vi "TrajectoryUtil_toPathWeaverJSON.vi"(7 "AlwaysOverWrite":bool, 8 "error in (no error)":errorcluster, 10 "inTRAJECTORY":T1 {"States"."POSE"."ROTATION"."SIN" format="%13.4f"; "States"."POSE"."ROTATION"."COS" format="%13.4f"; "States"."POSE"."ROTATION"."VALUE" format="%13.4f"; "States"."POSE"."TRANSLATION"."Y" format="%14.3f"; "States"."POSE"."TRANSLATION"."X" format="%14.3f"; "TotalTImeSecs" format="%20.3f"}, 11 "FileName":string="trajectory.json") -> (0 "error out":errorcluster, 4 "Full Filename":string)   [LabVIEW 2019, in "Trajectory_Library.lvlib"]
doc: "Exports a Trajectory to a PathWeaver-style JSON file.\n\nParameters:\n - Always Overwrite -- This optional terminal, if TRUE, will not prompt on WINDOWS to overwrite an existing file. On the RoboRIO the file is always overwritten. ( Default: False )\n - Trajectory - Trajectory data structure\n - FileName - File name string of the export json file\n - Error In - Error cluster (not used)\n\nReturns:\n - Error out - Returned error cluster"
uses:
  Trajectory_Library.lvlib
  TypeDef/TRAJECTORY.ctl
  TypeDef/TRAJ_STATE.ctl
  TypeDef/POSE2D.ctl
  TypeDef/TRANSLATION2D.ctl
  TypeDef/ROTATION2D.ctl
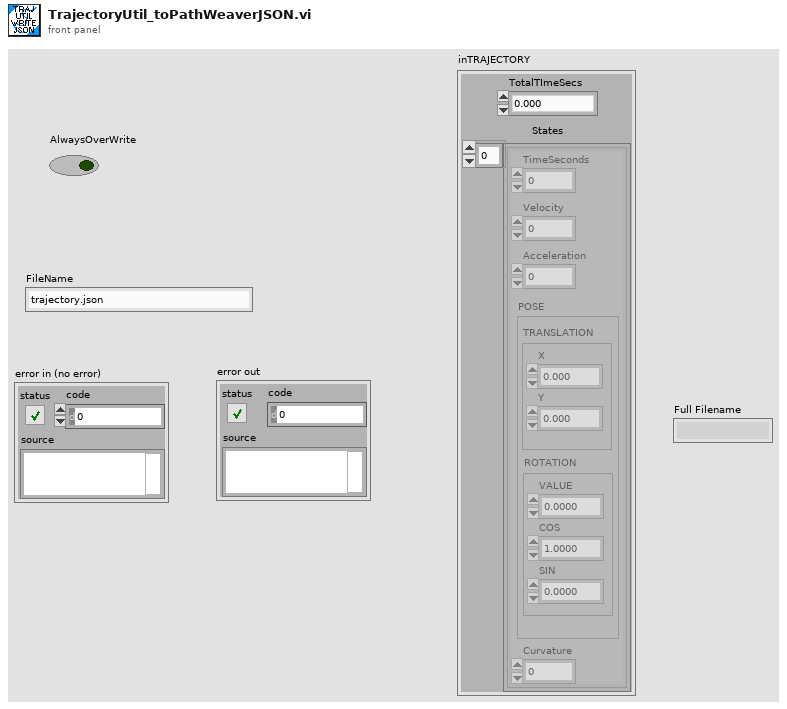
[diagram p1: front panel]
types:
  T1 = typedef "Trajectory_Library.lvlib/TRAJECTORY.ctl" = cluster{"TotalTImeSecs":dbl, "States":T2[]}
  T2 = typedef "Trajectory_Library.lvlib/TRAJ_STATE.ctl" = cluster{"TimeSeconds":dbl, "Velocity":dbl, "Acceleration":dbl, "POSE":T3, "Curvature":dbl}
  T3 = typedef "Trajectory_Library.lvlib/POSE2D.ctl" = cluster{"TRANSLATION":T4, "ROTATION":T5}
  T4 = typedef "Trajectory_Library.lvlib/TRANSLATION2D.ctl" = cluster{"X":dbl, "Y":dbl}
  T5 = typedef "Trajectory_Library.lvlib/ROTATION2D.ctl" = cluster{"VALUE":dbl, "COS":dbl, "SIN":dbl}
  T6 = enum16{"open", "replace", "create", "open or create", "replace or create", "replace or create with confirmation"}
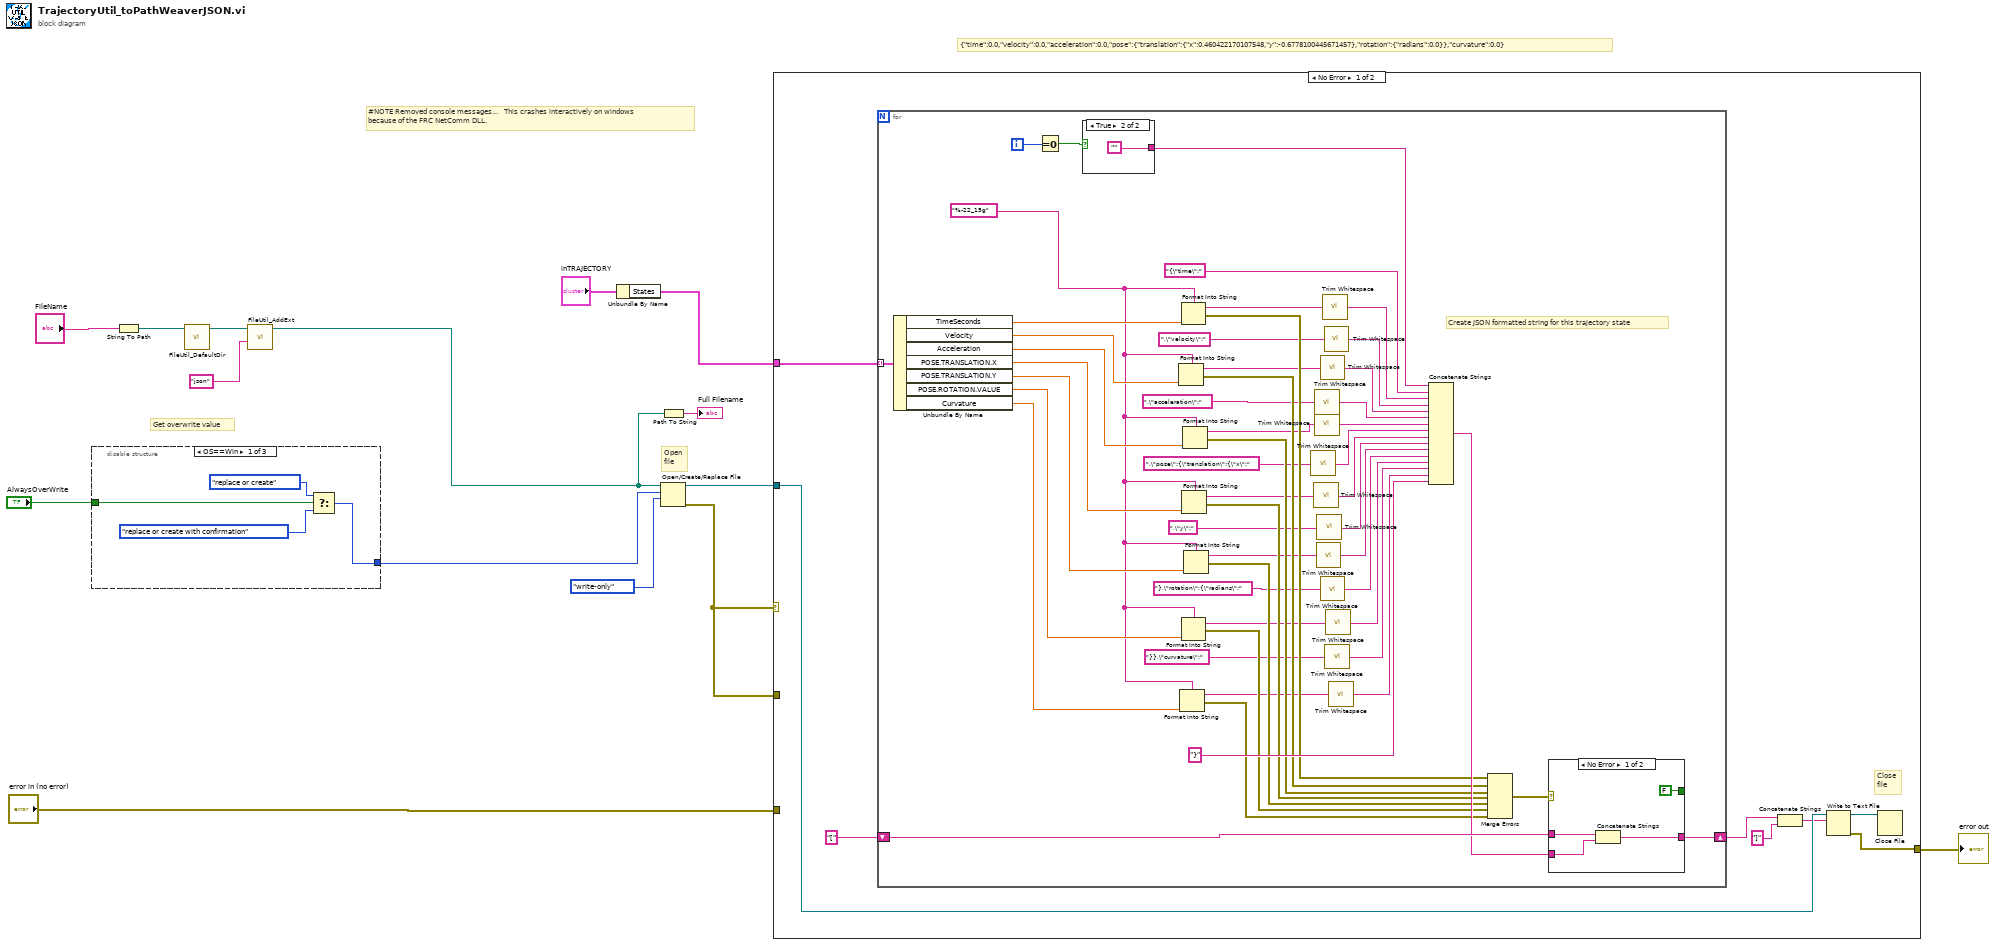
[diagram p0: block diagram]
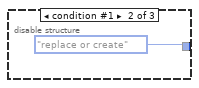
[diagram p2: hidden frame]
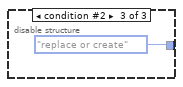
[diagram p3: hidden frame]
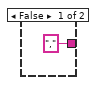
[diagram p4: hidden frame]
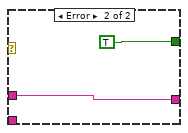
[diagram p5: hidden frame]
diagram:
  # "Get overwrite value"
  # "#NOTE Removed console messages...   This crashes interactively on windows \nbecause of the FRC NetComm DLL."
  # "{\"time\":0.0,\"velocity\":0.0,\"acceleration\":0.0,\"pose\":{\"translation\":{\"x\":0.460422170107548,\"y\":-0.6778100445671457},\"rotation\":{\"radians\":0.0}},\"curvature\":0.0}"
  # "Open\nfile"
  n1 = disable-structure shown="OS==Win" {
    disable-tunnel: [w16 T6."replace or create" ("operation (0:open)") T6."replace or create" ("operation (0:open)")] -> w8
    disable-tunnel: "AlwaysOverWrite" -> [w19 _ _]
    frame condition #0 (active) {
      n2 = Select(t=T6."replace or create" ("operation (0:open)"), s=w19, f=T6."replace or create with confirmation" ("operation (0:open)")) -> (s? t:f=w16:T6)
    }
    frame condition #1 {
    }
    frame condition #2 {
    }
  }
  n3 = String To Path(string="FileName") -> (path=w2:path)
  n4 = call "FileUtil_DefaultDir.vi"("Path in"=w2) -> ("Path Out"=w4:path)  [unwired: 10 in]
  n5 = call "FileUtil_AddExt.vi"("Extension"="json", "Path in"=w4) -> ("Path out"=w1:path)  [unwired: 9 in]
  n6 = Unbundle By Name("inTRAJECTORY") -> ("States"=w10:T2[])
  n7 = Open/Create/Replace File(file path (use dialog)=w1, operation (0:open)=w8, access (0:read/write)=enum16{"read/write", "read-only", "write-only"}."write-only") -> (refnum out=w9:refnum<file>, error out=w14:errorcluster)  [unwired: 3 in, 1 out]
  n8 = Path To String(path=w1) -> (string=→"Full Filename":string)
  n9 = case shown="No Error" w14 {
    tunnel: w14 -> [_ w89]
    tunnel: [w23 w89] -> w13
    tunnel: w10 -> [w29 _]
    tunnel: w9 -> [w25 _]
    tunnel: "error in (no error)" -> [_ _]
    frame No Error {
      # "Close\nfile"
      n10 = for {
        tunnel: w29 -> [w79] mode=indexing
        shift-right: [w65] -> w27
        shift-left: "[" -> [w66]
        i -> [w78]
        w56 = "%-22_15g"
        # "Create JSON formatted string for this trajectory state"
        n11 = Unbundle By Name(w79) -> ("TimeSeconds"=w73:dbl, "Velocity"=w72:dbl, "Acceleration"=w71:dbl, "POSE.TRANSLATION.X"=w70:dbl, "POSE.TRANSLATION.Y"=w69:dbl, "POSE.ROTATION.VALUE"=w68:dbl, "Curvature"=w67:dbl)
        n12 = Equal To 0?(x=w78) -> (x = 0?=w77:bool)
        n13 = case shown="True" w77 {
          tunnel: ["," ""] -> w76
          frame False {
          }
          frame True {
          }
        }
        n14 = Format Into String(format string=w56, w72) -> (resulting string=w51:string, error out=w62:errorcluster)  [unwired: 2 in]
        n15 = Format Into String(format string=w56, w67) -> (resulting string=w31:string, error out=w57:errorcluster)  [unwired: 2 in]
        n16 = Format Into String(format string=w56, w73) -> (resulting string=w55:string, error out=w63:errorcluster)  [unwired: 2 in]
        n17 = Format Into String(format string=w56, w68) -> (resulting string=w35:string, error out=w58:errorcluster)  [unwired: 2 in]
        n18 = Format Into String(format string=w56, w70) -> (resulting string=w43:string, error out=w60:errorcluster)  [unwired: 2 in]
        n19 = Format Into String(format string=w56, w71) -> (resulting string=w47:string, error out=w61:errorcluster)  [unwired: 2 in]
        n20 = Format Into String(format string=w56, w69) -> (resulting string=w39:string, error out=w59:errorcluster)  [unwired: 2 in]
        n21 = call <vilib>:"Trim Whitespace.vi"("string"=",\"pose\":{\"translation\":{\"x\":") -> ("trimmed string"=w44:string)  [unwired: 1 in]
        n22 = call <vilib>:"Trim Whitespace.vi"("string"=w43) -> ("trimmed string"=w42:string)  [unwired: 1 in]
        n23 = call <vilib>:"Trim Whitespace.vi"("string"=",\"acceleration\":") -> ("trimmed string"=w48:string)  [unwired: 1 in]
        n24 = call <vilib>:"Trim Whitespace.vi"("string"=w47) -> ("trimmed string"=w46:string)  [unwired: 1 in]
        n25 = call <vilib>:"Trim Whitespace.vi"("string"=w39) -> ("trimmed string"=w38:string)  [unwired: 1 in]
        n26 = call <vilib>:"Trim Whitespace.vi"("string"=",\"y\":") -> ("trimmed string"=w40:string)  [unwired: 1 in]
        n27 = call <vilib>:"Trim Whitespace.vi"("string"=w51) -> ("trimmed string"=w50:string)  [unwired: 1 in]
        n28 = call <vilib>:"Trim Whitespace.vi"("string"="},\"rotation\":{\"radians\":") -> ("trimmed string"=w36:string)  [unwired: 1 in]
        n29 = call <vilib>:"Trim Whitespace.vi"("string"=w55) -> ("trimmed string"=w54:string)  [unwired: 1 in]
        n30 = call <vilib>:"Trim Whitespace.vi"("string"=",\"velocity\":") -> ("trimmed string"=w52:string)  [unwired: 1 in]
        n31 = call <vilib>:"Trim Whitespace.vi"("string"="}},\"curvature\":") -> ("trimmed string"=w32:string)  [unwired: 1 in]
        n32 = call <vilib>:"Trim Whitespace.vi"("string"=w35) -> ("trimmed string"=w34:string)  [unwired: 1 in]
        n33 = call <vilib>:"Trim Whitespace.vi"("string"=w31) -> ("trimmed string"=w30:string)  [unwired: 1 in]
        n34 = Concatenate Strings(w76, "{\"time\":", w54, w52, w50, w48, w46, w44, w42, w40, w38, w36, w34, w32, w30, "}") -> (w64:string)
        n35 = Merge Errors(w63, w62, w61, w60, w59, w58, w57) -> (w80:errorcluster)
        n36 = case shown="No Error" w80 {
          tunnel: [FALSE TRUE] -> _
          tunnel: w66 -> [w85 w87]
          tunnel: [w84 w87] -> w65
          tunnel: w64 -> [w83 _]
          frame No Error {
            n37 = Concatenate Strings(w85, w83) -> (w84:string)
          }
          frame Error {
          }
        }
      }
      n38 = Concatenate Strings(w27, "]" ("string")) -> (w24:string)
      n39 = Write to Text File(file (use dialog)=w25, text=w24) -> (refnum out=w22:refnum<file>, error out=w23:errorcluster)  [unwired: 2 in, 1 out]
      n40 = Close File(refnum=w22) -> ()  [unwired: 1 in, 2 out]
    }
    frame Error {
      # "#NOTE Removed send error."
    }
  }
  "error out" <- w13
